vi "Define Columns.vi"() -> (2 "Column Definition":T1[](array[typedef]) {"MinWidth" min=2 step=1; "AutoSizeMode" items=["None"=1, "ColumnHeader"=2, "AllCellsExceptHeader"=4, "AllCells"=6, "DisplayedCellsExceptHeader"=8, "DisplayedCells"=10, "Fill"=16]; "FillWeight" min=1 max=100})   [LabVIEW 2015, in "DAQmx Module editor node.lvclass"]
doc: "This VI defines the columns that will be used in the table. You can specify the column type and the dimensions if the columns."
uses:
  DAQmx Module editor node.lvclass
  <vilib>/NI/DCAF/Tag Editor Core/Table API/Column/Column Descriptor.ctl
  <vilib>/NI/DCAF/Tag Editor Core/Table API/Column/Column.lvclass
  <vilib>/NI/DCAF/Tag Editor Core/Table API/Column/Column Type.ctl
  <vilib>/NI/Tag Bus/tag/Data Type.ctl
  <vilib>/NI/DCAF/Tag Editor Core/Table API/Table Manager/Call Back Ref Type Def.ctl
  <vilib>/NI/DCAF/Tag Editor Core/Configuration Editor/Classes/Engine Parent/Engine Parent Editor Node.lvclass
  <vilib>/NI/DCAF/Tag Editor Core/Configuration Editor/Classes/Module editor node/module editor node.lvclass
  <vilib>/NI/DCAF/Tag Editor Core/Table API/String Column/String Column.lvclass
  <vilib>/NI/DCAF/Tag Editor Core/Table API/Mapping Column/Mapping Column.lvclass
  <vilib>/NI/Tag Bus/tag/tag descriptor.lvclass
  <vilib>/NI/DCAF/Tag Editor Core/Table API/Table Manager/Table Manager.lvclass
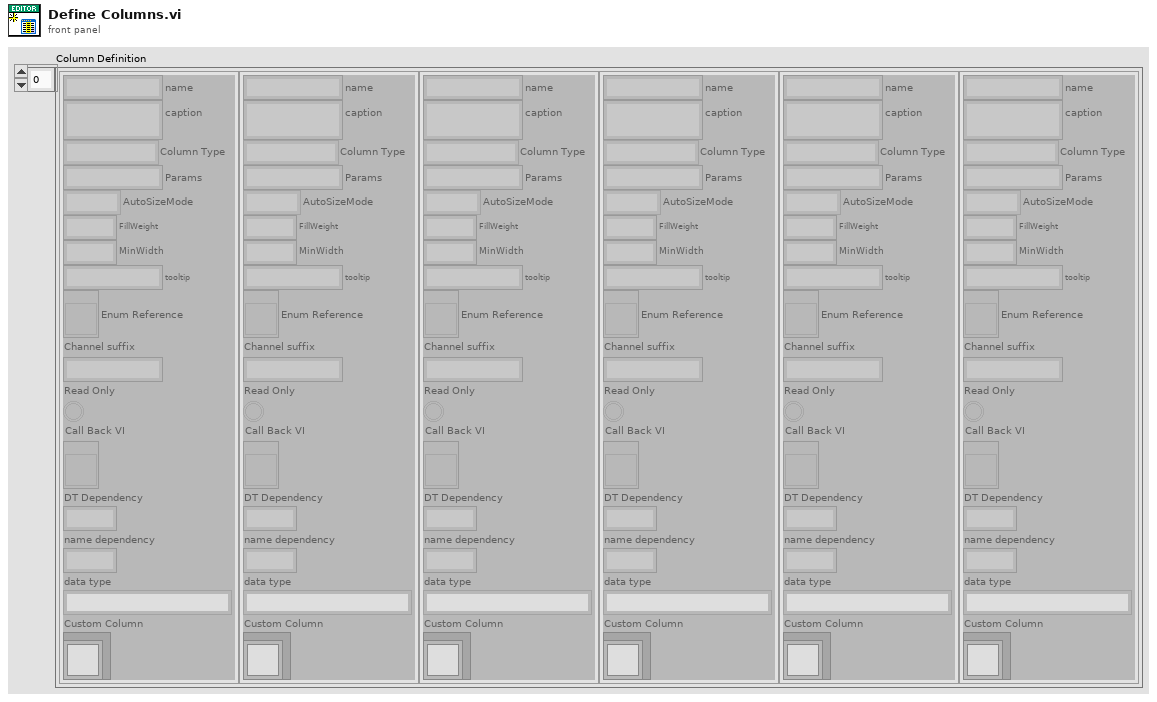
[diagram p1: front panel]
types:
  T1 = typedef "Table Manager.lvlib/Column.lvclass/Column Descriptor.ctl" = cluster{"name":string, "caption":string, "Column Type":T2, "Params":string, "AutoSizeMode":i32, "FillWeight":sgl, "MinWidth":u32, "tooltip":string, "Enum Reference":refnum<vi>, "Channel suffix":string, "Read Only":bool, "Call Back VI":T3, "DT Dependency":i32, "name dependency":i32, "data type":T4, "Custom Column":refnum<class "Column.lvclass">}
  T2 = typedef "Table Manager.lvlib/Column.lvclass/Column Type.ctl" = enum16{"String", "Mapping", "Enum", "Custom"}
  T3 = typedef "Table Manager.lvlib/Table Manager.lvclass/Call Back Ref Type Def.ctl" = refnum<vi>
  T4 = typedef "tag bus.lvlib/tag descriptor.lvclass/Data Type.ctl" = enum16{"Double", "Single", "I64", "I32", "I16", "I8", "U64", "U32", "U16", "U8", "Boolean", "String", "Array of Double", "Array of Single", "Array of I64", "Array of I32", "Array of I16", "Array of I8", "Array of U64", "Array of U32", "Array of U16", "Array of U8", "Array of Boolean", "Array of String"}
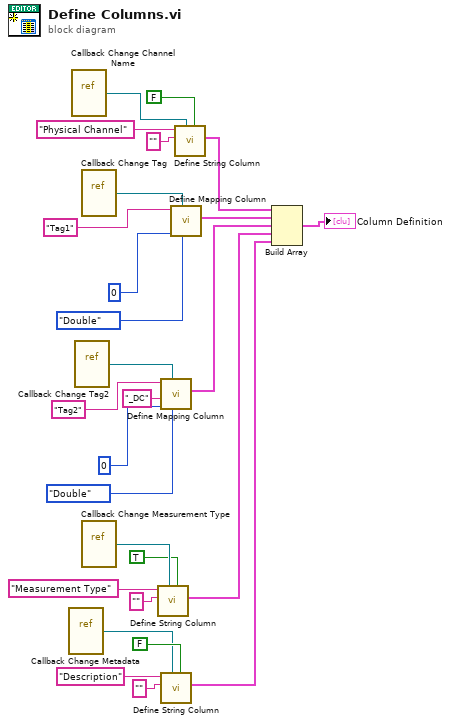
[diagram p0: block diagram]
diagram:
  n1 = vi-ref "Callback Change Metadata.vi"() -> (w8:refnum<vi>)
  n2 = vi-ref "Callback Change Channel Name.vi"() -> (w9:refnum<vi>)
  n3 = vi-ref "Callback Change Tag2.vi"() -> (w3:refnum<vi>)
  n4 = vi-ref "Callback Change Tag.vi"() -> (w27:refnum<vi>)
  n5 = vi-ref "Callback Change Measurement Type.vi"() -> (w11:refnum<vi>)
  n6 = call <vilib>:"Define String Column.vi"("Read Only (F)"=TRUE ("Read Only"), "Call Back VI"=w11, "Caption"="", "Name"="Measurement Type" ("name")) -> ("Column Descriptor out"=w7:T1)  [unwired: 7 in]
  n7 = call <vilib>:"Define Mapping Column.vi"("data type"=Data_Type."Double", "Call Back VI"=w3, "name dependency"=0, "Channel suffix"="_DC", "name"="Tag2") -> ("Column Descriptor out"=w2:T1)  [unwired: 6 in]
  n8 = call <vilib>:"Define String Column.vi"("Read Only (F)"=FALSE ("Read Only"), "Call Back VI"=w8, "Caption"="", "Name"="Description" ("name")) -> ("Column Descriptor out"=w14:T1)  [unwired: 7 in]
  n9 = call <vilib>:"Define Mapping Column.vi"("data type"=Data_Type."Double", "Call Back VI"=w27, "name dependency"=0, "name"="Tag1") -> ("Column Descriptor out"=w19:T1)  [unwired: 7 in]
  n10 = call <vilib>:"Define String Column.vi"("Read Only (F)"=FALSE ("Read Only"), "Call Back VI"=w9, "Caption"="", "Name"="Physical Channel" ("name")) -> ("Column Descriptor out"=w15:T1)  [unwired: 7 in]
  n11 = Build Array(w15, w19, w2, w7, w14) -> (→"Column Definition":T1[])
